vi "OwnOop20261013_CreateAccessorsDetached.vi"() -> ()   [LabVIEW 2024]
uses:
  <resource>/Framework/Providers/LVClassLibrary/NewAccessors/MemberVICreation.lvlib
panel:
  out "error out":errorcluster caption="错误输出"
  in  "Save Class Path":path
  in  "Write Path Without Diagram":bool
  in  "Write Path Save a Copy":bool
  in  "Write Path":path
  in  "Read Path Without Diagram":bool
  in  "Read Path Save a Copy":bool
  in  "Read Path":path
  in  "Virtual Folder Name":string
  in  "PDC Item Refnum":refnum<vi>
  in  "Make available through Property Nodes":bool
  in  "Include error terminals":bool
  in  "Access UI":enum16{"Read", "Write", "R/W"}(ring)
  in  "VI Type":enum32{"Dynamic", "Static"}(ring)=enum."Static"
  in  "Class Path":path
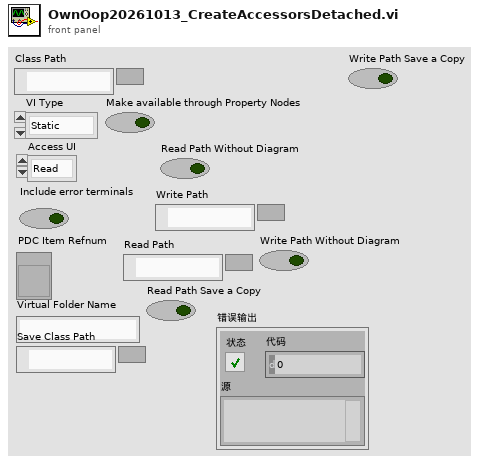
[diagram p1: front panel]
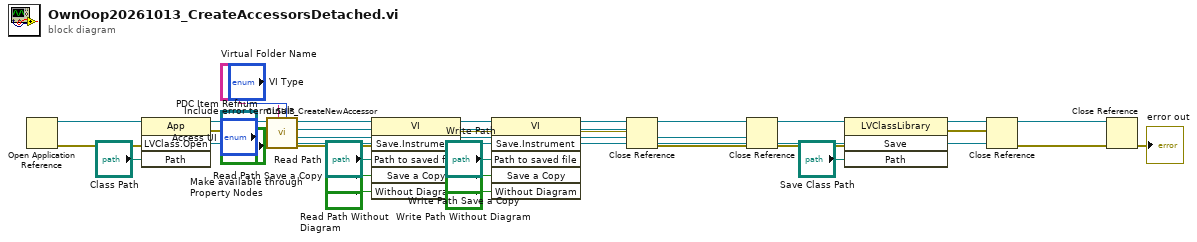
[diagram p0: block diagram]
diagram:
  n1 = Open Application Reference() -> (0:w26:errorcluster, 3:w28:refnum<vi>)  [unwired: 4 in]
  n2 = invoke class="App" method="LVClass.Open"(reference=w28, error in=w26, "Path"="Class Path") -> (error out=w24:errorcluster, "LVClass.Open"=w25:refnum<vi>)  [unwired: 1 in, 2 out]
  n3 = call <resource>:"CLSUIP_CreateNewAccessor.vi"("Make available through Property Nodes"="Make available through Property Nodes", "VI Type"="VI Type", "Include error terminals"="Include error terminals", "Virtual Folder Name"="Virtual Folder Name", "error in (no error)"=w24, "Access UI"="Access UI", "PDC Item Refnum"="PDC Item Refnum", "LVClassLibrary Ref"=w25) -> ("error out"=w13:errorcluster, "Write VI"=w12:refnum<vi>, "Read VI"=w17:refnum<vi>)  [unwired: 1 in]
  n4 = invoke class="VI" method="Save.Instrument"(reference=w17, error in=w13, "Path to saved file"="Read Path", "Save a Copy"="Read Path Save a Copy", "Without Diagram"="Read Path Without Diagram") -> (error out=w8:errorcluster)  [unwired: 1 in, 5 out]
  n5 = invoke class="VI" method="Save.Instrument"(reference=w12, error in=w8, "Path to saved file"="Write Path", "Save a Copy"="Write Path Save a Copy", "Without Diagram"="Write Path Without Diagram") -> (error out=w7:errorcluster)  [unwired: 1 in, 5 out]
  n6 = Close Reference(reference=w17, error in (no error)=w7) -> (error out=w6:errorcluster)
  n7 = Close Reference(reference=w12, error in (no error)=w6) -> (error out=w4:errorcluster)
  n8 = invoke class="LVClassLibrary" method="Save"(reference=w25, error in=w4, "Path"="Save Class Path") -> (error out=w3:errorcluster)  [unwired: 1 in, 3 out]
  n9 = Close Reference(reference=w25, error in (no error)=w3) -> (error out=w2:errorcluster)
  n10 = Close Reference(reference=w28, error in (no error)=w2) -> (error out=→"error out":errorcluster)
